vi "test for CP check.vi"(8 "CP A Tag AZ":string[](array[string]), 11 "CP Profile Table for RSeq":string[][](table)) -> (0 "LAP_Tag":string[](array[string]), 3 "Base Table RSeq":string[][](table) caption="CP Profile Table for RSeq")   [LabVIEW 2018]
panel:
  out "Signal Intensity [pA]":string[](array[string])
  out "subarray":string[](array[string])
  out "Relative Assigned Level":string[](array[string])
  out "Relative Assigned Level":string[](array[string])
  out "Base Time length [ms]":dbl[](array[numeric])
  out "CP Length [ms]":string[](array[string])
  out "Assigned Base":string[](array[string])
  out "Assigned Base":string[](array[string])
  out "S#":string[](array[string])
  out "number":i32[](array[numeric])
  out "Direction":string[](array[string])
  out "Relative Averaged Data":string[](array[string])
  out "MS_IDX":string[](array[string])
  out "L#":string[](array[string])
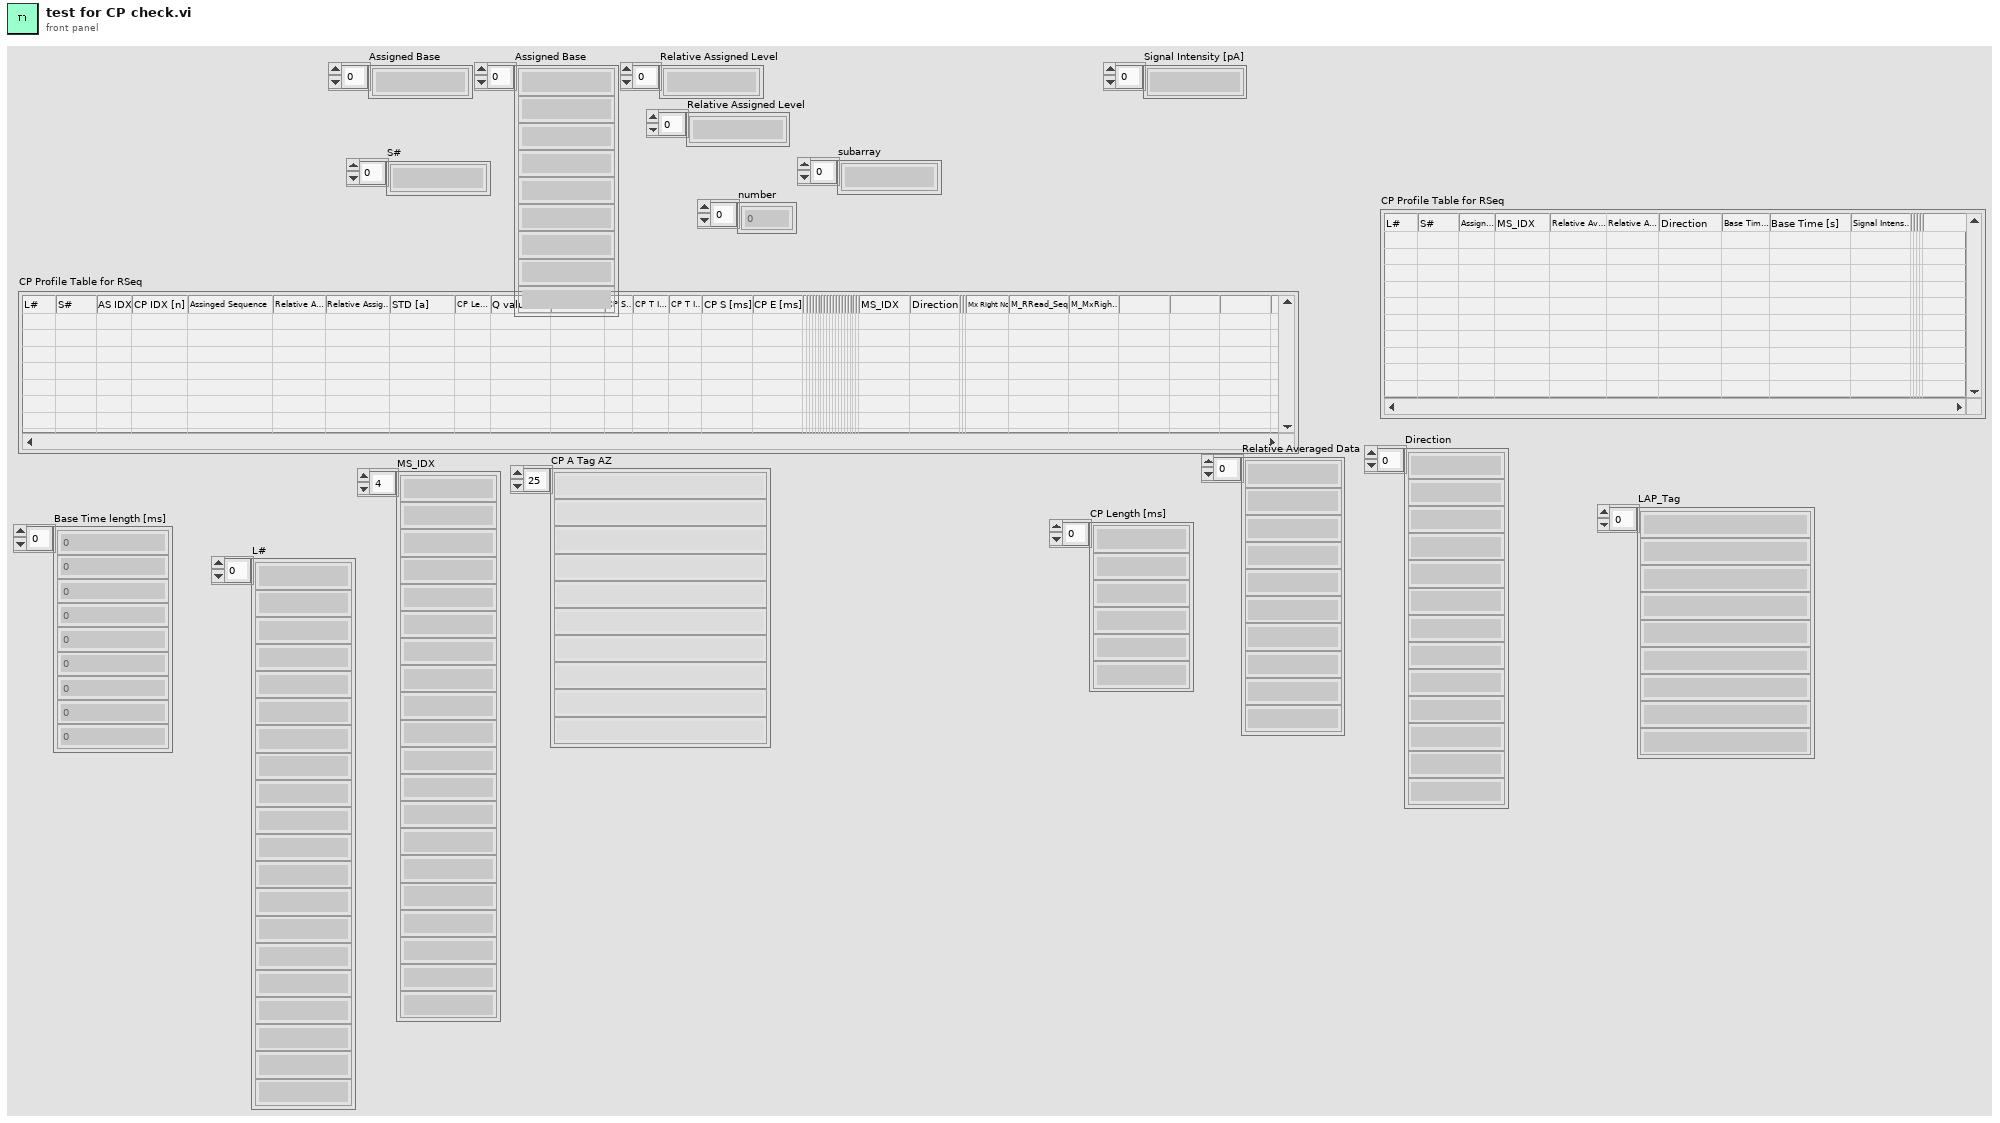
[diagram p1: front panel]
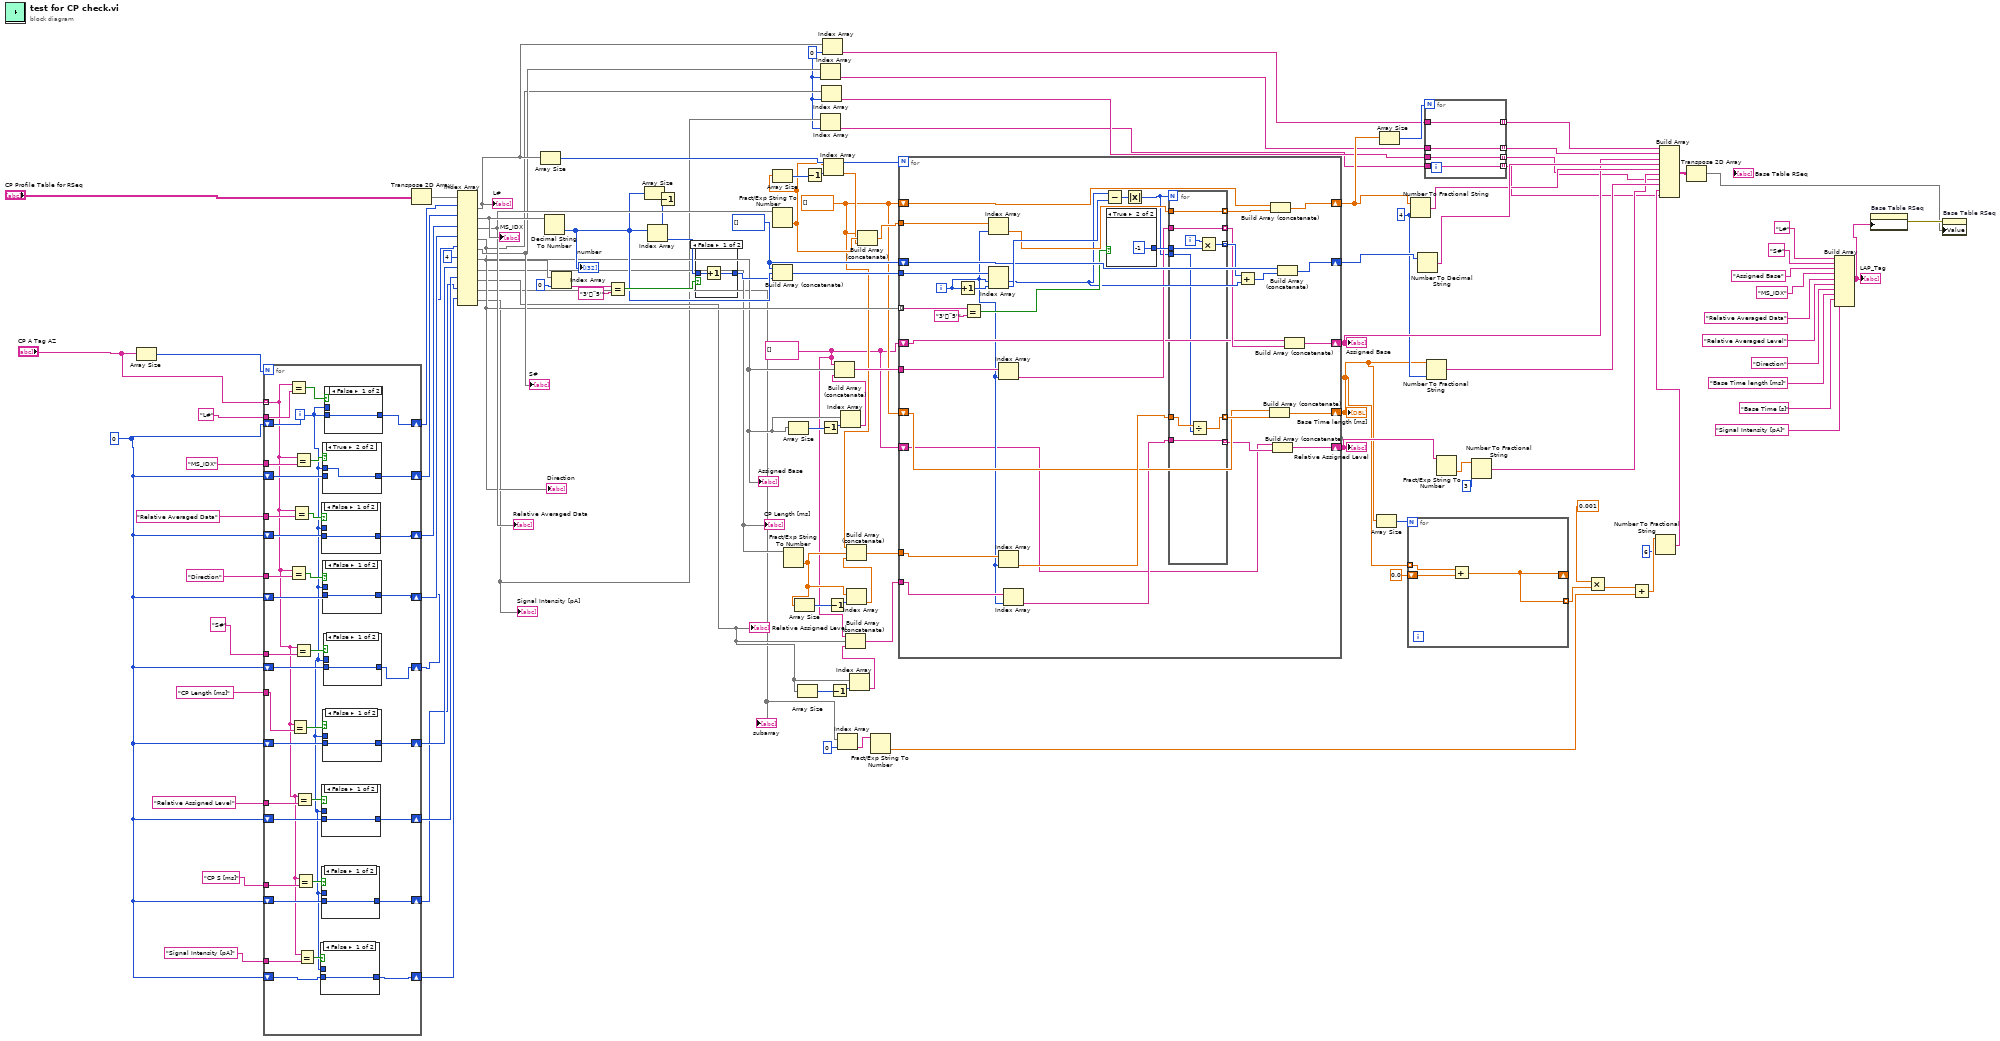
[diagram p0: block diagram]
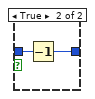
[diagram p11: hidden frame]
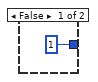
[diagram p12: hidden frame]
diagram:
  w39 = i16 4 ("precision (6)")
  w43 = string[] []
  w4 = 0 ("index")
  w7 = 0 ("index (row)")
  w102 = i32[] []
  w54 = dbl[] []
  n1 = Array Size(array="CP A Tag AZ") -> (size(s)=w92:i32)
  n2 = for {
    N: w92 -> [_]
    tunnel: "CP A Tag AZ" -> [w119] mode=indexing
    tunnel: "L#" ("y") -> [w151]
    shift-right: [w149] -> w86
    shift-left: w7 -> [w150]
    shift-right: [w146] -> w85
    shift-left: w7 -> [w147]
    shift-right: [w144] -> w84
    shift-left: w7 -> [w145]
    shift-right: [w142] -> w83
    shift-left: w7 -> [w143]
    tunnel: "MS_IDX" ("y") -> [w140]
    tunnel: "Relative Averaged Data" ("y") -> [w139]
    tunnel: "Direction" ("y") -> [w138]
    tunnel: "S#" ("y") -> [w134]
    shift-right: [w133] -> w81
    shift-left: w7 -> [w132]
    shift-right: [w130] -> w61
    shift-left: w7 -> [w131]
    tunnel: "CP Length [ms]" ("y") -> [w129]
    tunnel: "Relative Assigned Level" ("y") -> [w126]
    shift-right: [w124] -> w49
    shift-left: w7 -> [w125]
    shift-right: [w122] -> w36
    shift-left: w7 -> [w121]
    tunnel: "CP S [ms]" ("y") -> [w120]
    shift-right: [w115] -> w6
    shift-left: w7 -> [w114]
    tunnel: "Signal Intensity [pA]" ("y") -> [w117]
    i -> [w116]
    n3 = Equal?(x=w119, y=w151) -> (x = y?=w148:bool)
    n4 = Equal?(x=w119, y=w138) -> (x = y?=w136:bool)
    n5 = Equal?(x=w119, y=w129) -> (x = y?=w128:bool)
    n6 = Equal?(x=w119, y=w139) -> (x = y?=w137:bool)
    n7 = Equal?(x=w119, y=w140) -> (x = y?=w141:bool)
    n8 = Equal?(x=w119, y=w134) -> (x = y?=w135:bool)
    n9 = Equal?(x=w119, y=w126) -> (x = y?=w127:bool)
    n10 = Equal?(x=w119, y=w120) -> (x = y?=w123:bool)
    n11 = Equal?(x=w119, y=w117) -> (x = y?=w118:bool)
    n12 = case shown="False" w118 {
      tunnel: w116 -> [_ w153]
      tunnel: [w152 w153] -> w115
      tunnel: w114 -> [w152 _]
      frame False {
      }
      frame True {
      }
    }
    n13 = case shown="False" w123 {
      tunnel: w116 -> [_ w155]
      tunnel: [w154 w155] -> w122
      tunnel: w121 -> [w154 _]
      frame False {
      }
      frame True {
      }
    }
    n14 = case shown="False" w137 {
      tunnel: w116 -> [_ w165]
      tunnel: [w164 w165] -> w144
      tunnel: w145 -> [w164 _]
      frame False {
      }
      frame True {
      }
    }
    n15 = case shown="False" w127 {
      tunnel: w116 -> [_ w157]
      tunnel: [w156 w157] -> w124
      tunnel: w125 -> [w156 _]
      frame False {
      }
      frame True {
      }
    }
    n16 = case shown="True" w141 {
      tunnel: w116 -> [_ w167]
      tunnel: [w166 w167] -> w146
      tunnel: w147 -> [w166 _]
      frame False {
      }
      frame True {
      }
    }
    n17 = case shown="False" w136 {
      tunnel: w116 -> [_ w163]
      tunnel: [w162 w163] -> w142
      tunnel: w143 -> [w162 _]
      frame False {
      }
      frame True {
      }
    }
    n18 = case shown="False" w128 {
      tunnel: w116 -> [_ w159]
      tunnel: [w158 w159] -> w130
      tunnel: w131 -> [w158 _]
      frame False {
      }
      frame True {
      }
    }
    n19 = case shown="False" w135 {
      tunnel: w116 -> [_ w161]
      tunnel: [w160 w161] -> w133
      tunnel: w132 -> [w160 _]
      frame False {
      }
      frame True {
      }
    }
    n20 = case shown="False" w148 {
      tunnel: w116 -> [_ w169]
      tunnel: [w168 w169] -> w149
      tunnel: w150 -> [w168 _]
      frame False {
      }
      frame True {
      }
    }
  }
  n21 = Transpose 2D Array(2D array="CP Profile Table for RSeq") -> (transposed array=w112:string[][])
  n22 = Index Array(array=w112, index (row) #1=w86, index (row) #2=w85, index (row) #3=w84, index (row) #4=w83, index (row) #5=w81, index (row) #6=4 ("index (row)"), index (row) #7=w61, index (row) #8=w49, index (row) #9=w36, index (row) #10=w6) -> (element #1=w74:string[], element #2=w110:string[], element #3=w109:string[], element #4=w70:string[], element #5=w72:string[], element #6=w65:string[], element #7=w60:string[], element #8=w46:string[], element #9=w35:string[], element #10=w5:string[])  [unwired: 10 in]
  "L#" <- w74
  "MS_IDX" <- w110
  "Relative Averaged Data" <- w109
  "Direction" <- w70
  "S#" <- w72
  "Assigned Base" <- w65
  "CP Length [ms]" <- w60
  "Relative Assigned Level" <- w46
  "subarray" <- w35
  "Signal Intensity [pA]" <- w5
  n23 = Array Size(array=w74) -> (size(s)=w113:i32)
  n24 = Decimal String To Number(string=w110) -> (number=w98:i32[])  [unwired: 2 in, 1 out]
  "number" <- w98
  n25 = Index Array(array=w70, index=0) -> (element=w106:string)
  n26 = Equal?(x=w106, y="3'¨5'") -> (x = y?=w105:bool)
  n27 = Array Size(array=w98) -> (size(s)=w99:i32)
  n28 = Decrement(x=w99) -> (x-1=w96:i32)
  n29 = Index Array(array=w98, index=w96) -> (element=w104:i32)
  n30 = case shown="False" w105 {
    tunnel: w104 -> [w171 w173]
    tunnel: [w170 w172] -> w97
    frame False {
      n31 = Increment(x=w171) -> (x+1=w170:i32)
    }
    frame True {
      n32 = Decrement(x=w173) -> (x-1=w172:i32)
    }
  }
  n33 = Fract/Exp String To Number(string=w109) -> (number=w94:dbl[])  [unwired: 3 in, 1 out]
  n34 = Array Size(array=w94) -> (size(s)=w100:i32)
  n35 = Build Array (concatenate)(w102, w98, w97) -> (w103:i32[])
  n36 = Fract/Exp String To Number(string=w60) -> (number=w57:dbl[])  [unwired: 3 in, 1 out]
  n37 = Array Size(array=w65) -> (size(s)=w67:i32)
  n38 = Array Size(array=w57) -> (size(s)=w59:i32)
  n39 = Array Size(array=w46) -> (size(s)=w48:i32)
  n40 = Decrement(x=w100) -> (x-1=w95:i32)
  n41 = Index Array(array=w72, index=w4) -> (element=w71:string)
  n42 = Index Array(array=w5, index=w4) -> (element=w3:string)
  n43 = Decrement(x=w67) -> (x-1=w66:i32)
  n44 = Index Array(array=w70, index=w4) -> (element=w69:string)
  n45 = Index Array(array=w74, index=w4) -> (element=w73:string)
  n46 = Index Array(array=w94, index=w95) -> (element=w93:dbl)
  n47 = Decrement(x=w59) -> (x-1=w58:i32)
  n48 = Decrement(x=w48) -> (x-1=w47:i32)
  n49 = Index Array(array=w35, index=0) -> (element=w33:string)
  n50 = Index Array(array=w65, index=w66) -> (element=w64:string)
  n51 = Build Array (concatenate)(w43, w65, w64) -> (w63:string[])
  n52 = Index Array(array=w57, index=w58) -> (element=w56:dbl)
  n53 = Build Array (concatenate)(w54, w57, w56) -> (w55:dbl[])
  n54 = Index Array(array=w46, index=w47) -> (element=w45:string)
  n55 = Build Array (concatenate)(w43, w46, w45) -> (w44:string[])
  n56 = Build Array (concatenate)(w54, w94, w93) -> (w101:dbl[])
  n57 = Fract/Exp String To Number(string=w33) -> (number=w29:dbl)  [unwired: 3 in, 1 out]
  n58 = for {
    N: w113 -> [_]
    tunnel: w70 -> [w208] mode=indexing
    tunnel: w103 -> [w206]
    shift-right: [w203] -> w80
    shift-left: w102 -> [w202]
    shift-right: [w200] -> w79
    shift-left: w54 -> [w199]
    tunnel: w101 -> [w198]
    tunnel: w63 -> [w191]
    shift-right: [w188] -> w51
    shift-left: w43 -> [w187]
    tunnel: w55 -> [w186]
    shift-right: [w183] -> w31
    shift-left: w54 -> [w182]
    tunnel: w44 -> [w180]
    shift-right: [w176] -> w41
    shift-left: w43 -> [w175]
    i -> [w179]
    n59 = Increment(x=w179) -> (x+1=w205:i32)
    n60 = Equal?(x=w208, y="3'¨5'") -> (x = y?=w201:bool)
    n61 = Index Array(array=w198, index=w179) -> (element=w193:dbl)
    n62 = Index Array(array=w206, index #1=w179, index #2=w205) -> (element #1=w192:i32, element #2=w204:i32)
    n63 = Index Array(array=w191, index=w179) -> (element=w190:string)
    n64 = Index Array(array=w186, index=w179) -> (element=w185:dbl)
    n65 = Index Array(array=w180, index=w179) -> (element=w178:string)
    n66 = Subtract(x=w192, y=w204) -> (x-y=w181:i32)
    n67 = case shown="True" w201 {
      tunnel: [1 -1] -> w195
      frame False {
      }
      frame True {
      }
    }
    n68 = Absolute Value(x=w181) -> (abs(x)=w174:i32)
    n69 = for {
      N: w174 -> [_]
      tunnel: [w219] -> w196 mode=indexing
      tunnel: w195 -> [w218]
      tunnel: w193 -> [w216]
      tunnel: [w216] -> w194 mode=indexing
      tunnel: w190 -> [w215]
      tunnel: [w215] -> w189 mode=indexing
      tunnel: w185 -> [w214]
      tunnel: [w213] -> w184 mode=indexing
      tunnel: w174 -> [w212]
      tunnel: w178 -> [w211]
      tunnel: [w211] -> w177 mode=indexing
      i -> [w217]
      n70 = Divide(x=w214, y=w212) -> (x/y=w213:dbl)
      n71 = Multiply(x=w217, y=w218) -> (x*y=w219:i32)
    }
    n72 = Add(x=w196, y=w192) -> (x+y=w197:i32[])
    n73 = Build Array (concatenate)(w182, w184) -> (w183:dbl[])
    n74 = Build Array (concatenate)(w199, w194) -> (w200:dbl[])
    n75 = Build Array (concatenate)(w175, w177) -> (w176:string[])
    n76 = Build Array (concatenate)(w202, w197) -> (w203:i32[])
    n77 = Build Array (concatenate)(w187, w189) -> (w188:string[])
  }
  "Assigned Base" <- w51
  "Base Time length [ms]" <- w31
  "Relative Assigned Level" <- w41
  n78 = Array Size(array=w31) -> (size(s)=w32:i32)
  n79 = Array Size(array=w79) -> (size(s)=w78:i32)
  n80 = for {
    N: w32 -> [_]
    tunnel: w31 -> [w222] mode=indexing
    shift-right: [w220] -> _
    shift-left: 0.0 -> [w221]
    tunnel: [w220] -> w26 mode=indexing
    n81 = Add(x=w222, y=w221) -> (x+y=w220:dbl)
  }
  n82 = Number To Fractional String(number=w79, precision (6)=w39) -> (F-format string=w76:string[])  [unwired: 2 in]
  n83 = Number To Decimal String(number=w80) -> (decimal integer string=w77:string[])  [unwired: 1 in]
  n84 = for {
    N: w78 -> [_]
    tunnel: w73 -> [w226]
    tunnel: [w226] -> w53 mode=indexing
    tunnel: w71 -> [w225]
    tunnel: [w225] -> w52 mode=indexing
    tunnel: w69 -> [w224]
    tunnel: [w224] -> w14 mode=indexing
    tunnel: w3 -> [w223]
    tunnel: [w223] -> w2 mode=indexing
  }
  n85 = Number To Fractional String(number=w31, precision (6)=w39) -> (F-format string=w42:string[])  [unwired: 2 in]
  n86 = Fract/Exp String To Number(string=w41) -> (number=w40:dbl[])  [unwired: 3 in, 1 out]
  n87 = Number To Fractional String(number=w40, precision (6)=i16 3) -> (F-format string=w15:string[])  [unwired: 2 in]
  n88 = Multiply(x=0.001, y=w26) -> (x*y=w28:dbl[])
  n89 = Add(x=w28, y=w29) -> (x+y=w25:dbl[])
  n90 = Number To Fractional String(number=w25, precision (6)=i16 6) -> (F-format string=w23:string[])  [unwired: 2 in]
  n91 = Build Array(w53, w52, w51, w77, w76, w15, w14, w42, w23, w2) -> (w75:string[][])
  n92 = Transpose 2D Array(2D array=w75) -> (transposed array=w9:string[][])
  n93 = Build Array("L#" ("y"), "S#" ("y"), "Assigned Base" ("y"), "MS_IDX" ("y"), "Relative Averaged Data" ("y"), "Relative Averaged Level" ("y"), "Direction" ("y"), "Base Time length [ms]" ("y"), "Base Time [s]" ("y"), "Signal Intensity [pA]" ("y")) -> (w11:string[])
  "LAP_Tag" <- w11
  n94 = property on="Base Table RSeq" class="Tbl (strict)"("Column Headers[]"=w11) -> (error out=w10:errorcluster)  [unwired: 2 in, 1 out]
  n95 = property on="Base Table RSeq" class="Tbl (strict)"(error in=w10, "Value"=w9) -> ()  [unwired: 1 in, 2 out]
